vi "VITester_Global_OnCommand.vi"(10 "Command ID":string, 11 "Object":T1) -> ()   [LabVIEW 2013]
uses:
  Support/VITester Project Item Ref.ctl
panel:
  out "error out":errorcluster
  in  "error in":errorcluster
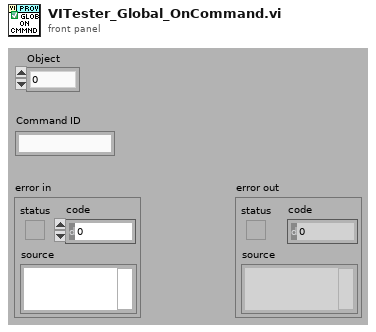
[diagram p1: front panel]
types:
  T1 = typedef "VITester Project Item Ref.ctl" = u64
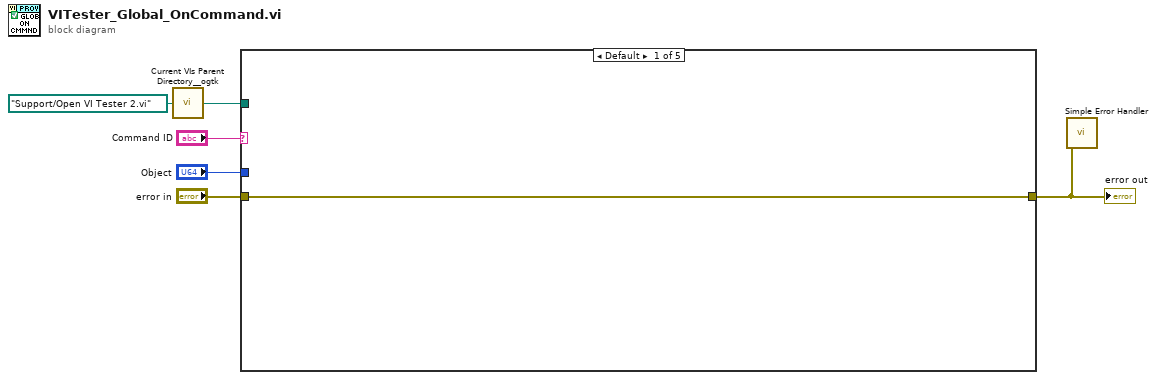
[diagram p0: block diagram]
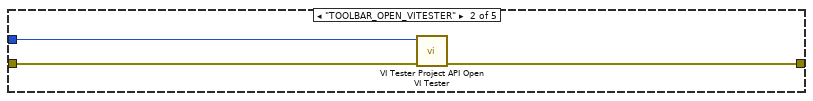
[diagram p2: hidden frame]
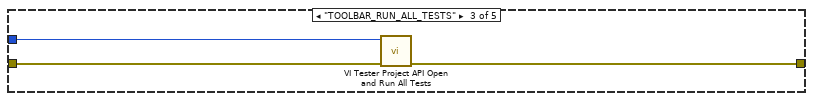
[diagram p3: hidden frame]
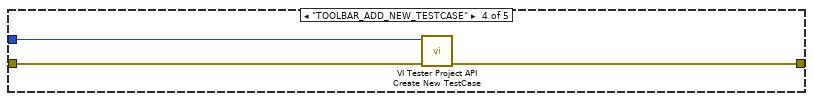
[diagram p4: hidden frame]
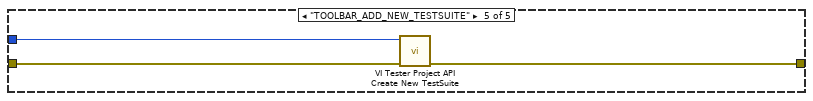
[diagram p5: hidden frame]
diagram:
  n1 = call <userlib>:"Current VIs Parent Directory__ogtk.vi"("Relative path (.)"=path "Support/Open VI Tester 2.vi") -> ("Parent Directory (+ Relative)"=w3:path)  [unwired: 4 in]
  n2 = case shown="Default" "Command ID" {
    tunnel: "error in" -> [w7 w10 w13 w15 w18]
    tunnel: [w7 w9 w11 w16 w19] -> w1
    tunnel: "Object" -> [_ w8 w12 w14 w17]
    tunnel: w3 -> [_ _ _ _ _]
    frame Default {
    }
    frame "TOOLBAR_OPEN_VITESTER" {
      n3 = call "VI Tester Project API Open VI Tester.vi"("error in"=w10, "Object"=w8) -> ("error out"=w9:errorcluster)  [unwired: 9 in]
    }
    frame "TOOLBAR_RUN_ALL_TESTS" {
      n4 = call "VI Tester Project API Open and Run All Tests.vi"("error in"=w13, "Object"=w12) -> ("error out"=w11:errorcluster)  [unwired: 9 in]
    }
    frame "TOOLBAR_ADD_NEW_TESTCASE" {
      n5 = call "VI Tester Project API Create New TestCase.vi"("error in"=w15, "Object"=w14) -> ("error out"=w16:errorcluster)  [unwired: 9 in]
    }
    frame "TOOLBAR_ADD_NEW_TESTSUITE" {
      n6 = call "VI Tester Project API Create New TestSuite.vi"("error in"=w18, "Object"=w17) -> ("error out"=w19:errorcluster)  [unwired: 9 in]
    }
  }
  "error out" <- w1
  n7 = call <vilib>:"Simple Error Handler.vi"("error in (no error)"=w1) -> ()  [unwired: 4 in, 5 out]
